vi "Check Full Name.vi"(8 "error in (no error)":errorcluster, 9 "Topic Name In":string, 11 "CIF_Iceoryx_BB in":refnum<class "CIF_Iceoryx_BB.lvclass">) -> (0 "error out":errorcluster, 2 "Topic Name out":string, 3 "Full Name Out":string)   [LabVIEW 2021, in "CIF_Iceoryx_BB.lvclass"]
uses:
  CIF_Iceoryx_BB.lvclass
  D:/dev/Packages/CIF_Channels_Core/src/CIFChannels/CIFChannels.lvclass
  CIFChannels/CIFChannels.lvclass/CIFChannels.ctl
  CIF_Iceoryx_Chan/Typedef/Iceoryx Channel Error.ctl
  CIF_Iceoryx_Chan/SubVIs/Iceoryx Channel Errors Core.vi
  CIFChannels/CIFChannels.lvclass
  Iceorxy Utilities/Iceoryx Channel Utilities.lvlib
  CIF_Iceoryx_Chan/CIF_Iceoryx_Chn.lvclass
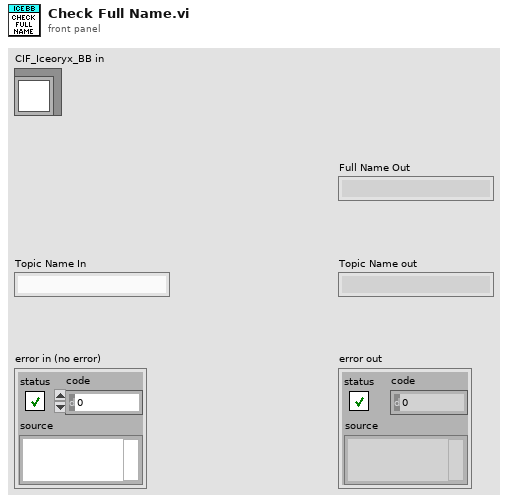
[diagram p1: front panel]
types:
  T1 = typedef "CIF_Iceoryx_Chn.lvclass/Iceoryx Channel Error.ctl" = enum16{"Type Mismatch", "Name Mismatch", "Override Required"}
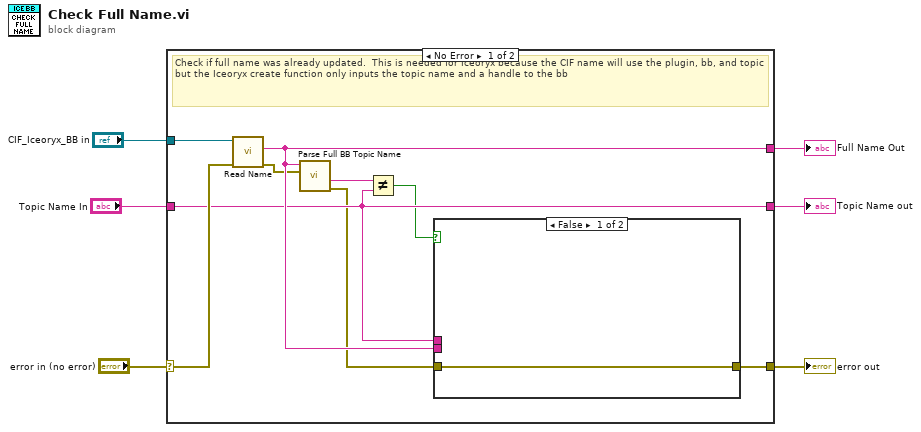
[diagram p0: block diagram]
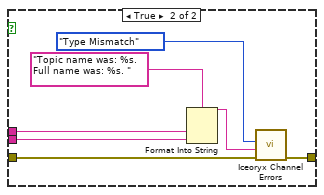
[diagram p2: hidden frame]
diagram:
  n1 = case shown="No Error" "error in (no error)" {
    selector: "error in (no error)" -> [w14 w25]
    tunnel: [w15 w25] -> w5
    tunnel: "CIF_Iceoryx_BB in" -> [w13 _]
    tunnel: "Topic Name In" -> [w11 w24]
    tunnel: [w12 w24] -> w2
    tunnel: [w11 w24] -> w1
    frame No Error {
      # "Check if full name was already updated.  This is needed for Iceoryx because the CIF name will use the plugin, bb, and topic but the Iceoryx create function only inputs the topic name and a handle to the bb"
      n2 = call "Read Name.vi"("error in (no error)"=w14, "CIFChannels in"=w13) -> ("error out"=w10:errorcluster, "Name"=w12:string)  [unwired: 7 in, 1 out]
      n3 = call "Parse Full BB Topic Name.vi"("error in"=w10, "Full BB Topic Name"=w12) -> ("error out"=w7:errorcluster, "Topic"=w9:string)  [unwired: 6 in, 2 out]
      n4 = Not Equal?(x=w9, y=w11) -> (x != y?=w8:bool)
      n5 = case shown="False" w8 {
        tunnel: [w16 w23] -> w15
        tunnel: w7 -> [w16 w22]
        tunnel: w11 -> [_ w19]
        tunnel: w12 -> [_ w20]
        frame False {
        }
        frame True {
          n6 = Format Into String(format string="Topic name was: %s.  Full name was: %s. ", w19, w20) -> (resulting string=w17:string)  [unwired: 2 in, 1 out]
          n7 = call "Iceoryx Channel Errors.vi"("error in (no error)"=w22, "String to Append"=w17, "Error"=Iceoryx_Channel_Error."Type Mismatch") -> ("error out"=w23:errorcluster)  [unwired: 8 in]
        }
      }
    }
    frame Error {
    }
  }
  "error out" <- w5
  "Topic Name out" <- w1
  "Full Name Out" <- w2
